vi "1.vi"() -> ()   [LabVIEW 2026]
panel:
  in  "Tab Control":enum32{"Hello", "Hai"}(tab)
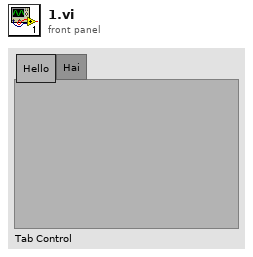
[diagram p1: front panel]
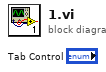
[diagram p0: block diagram]
diagram:
